vi "shear_cessation_voltage__62621484f0.vi"(7 "initial position in volt":dbl, 9 "shear cessation point":i32, 10 "amplitude":dbl=1.0 format="%0.2f", 11 "voltage to displacement contant":dbl) -> (3 "element":dbl)   [LabVIEW 2023]
uses:
  <vilib>/DAQmx/write.llb/DAQmx Write (Analog DBL 1Chan 1Samp).vi
  <vilib>/DAQmx/create/channels.llb/DAQmx Create Channel (AO-Voltage-Basic).vi
  <vilib>/DAQmx/miscellaneous.llb/DAQmx Fill In Error Info.vi
  <vilib>/Analysis/NI_AALBase.lvlib
panel:
  out "x+y":dbl[](array[numeric])
  out "Waveform Graph":dbl[](graph)
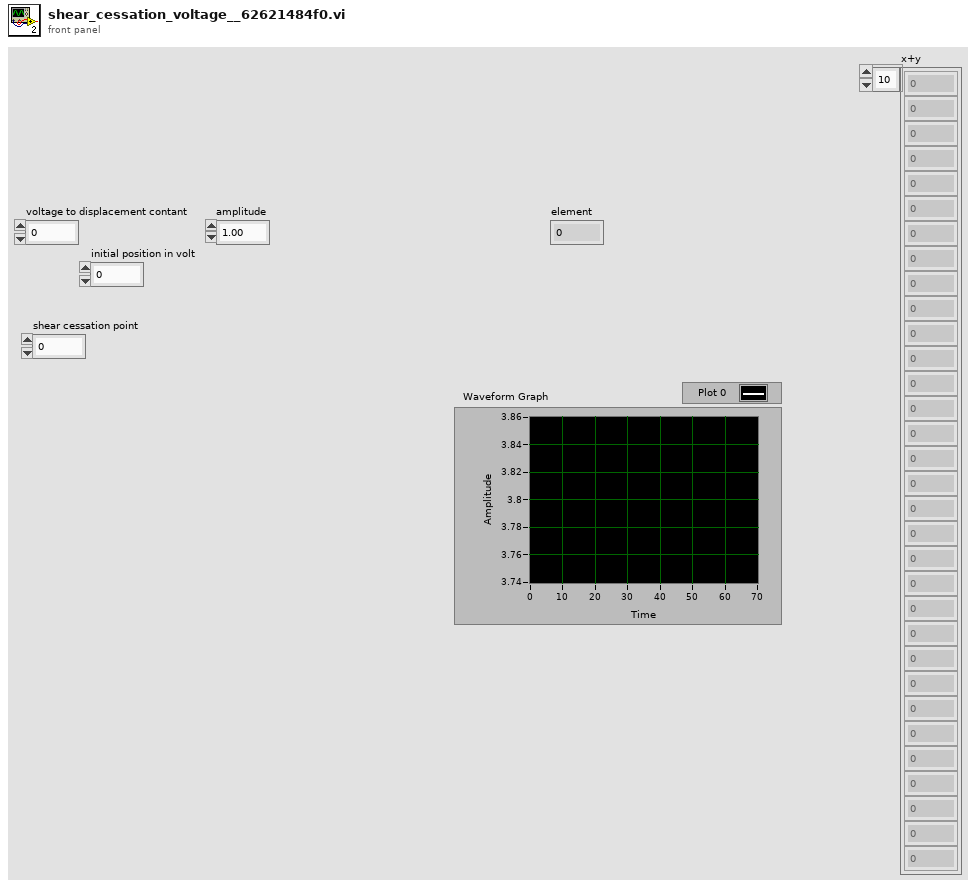
[diagram p1: front panel]
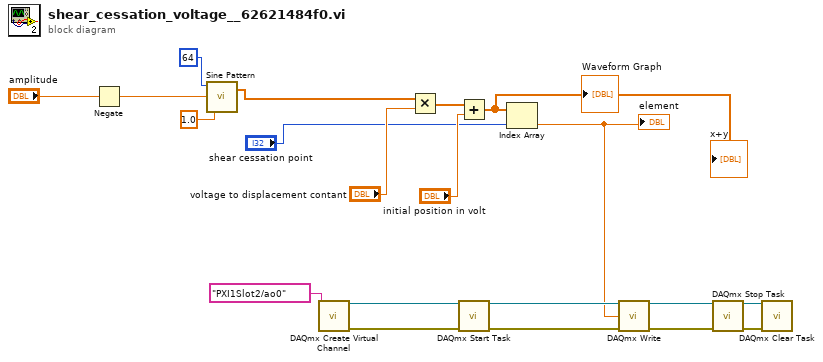
[diagram p0: block diagram]
diagram:
  n1 = Negate(x="amplitude") -> (-x=w1:dbl)
  n2 = call <vilib>:"Sine Pattern.vi"("cycles"=1.0, "amplitude"=w1, "samples"=64) -> ("Sinusoidal Pattern"=w15:dbl[])  [unwired: 1 in, 1 out]
  n3 = call-poly <vilib>:"DAQmx Create Virtual Channel.vi"("physical channels"=tag "PXI1Slot2/ao0") -> ("task out"=w10:refnum<k21>, "error out"=w11:errorcluster)  [unwired: 13 in]
  n4 = Multiply(x=w15, y="voltage to displacement contant") -> (x*y=w17:dbl[])
  n5 = Add(x=w17, y="initial position in volt") -> (x+y=w3:dbl[])
  "Waveform Graph" <- w3
  "x+y" <- w3
  n6 = call <vilib>:"DAQmx Start Task.vi"("task/channels in"=w10, "error in"=w11) -> ("task out"=w6:refnum<k21>, "error out"=w5:errorcluster)  [unwired: 12 in]
  n7 = Index Array(array=w3, index="shear cessation point") -> (element=w4:dbl)
  "element" <- w4
  n8 = call-poly <vilib>:"DAQmx Write.vi"("task/channels in"=w6, "data"=w4, "error in"=w5) -> ("task out"=w8:refnum<k21>, "error out"=w7:errorcluster)  [unwired: 10 in, 1 out]
  n9 = call <vilib>:"DAQmx Stop Task.vi"("task/channels in"=w8, "error in"=w7) -> ("task out"=w13:refnum<k21>, "error out"=w12:errorcluster)  [unwired: 12 in]
  n10 = call <vilib>:"DAQmx Clear Task.vi"("task in"=w13, "error in"=w12) -> ()  [unwired: 13 in, 1 out]
